vi "I2C Write Reg Block.vi"(8 "error in (no error)":errorcluster, 9 "Values":u8[](array[numeric]), 10 "Register":i32, 11 "I2C Device":T1) -> (0 "error out":errorcluster, 3 "I2C Device out":T1)   [LabVIEW 2020, in "wiringPi.lvlib"]
doc: "<b>_______________________________________________________________</b>\n** Author: Juan José Villacorta\n** LabVIEW wrapper for C library <b> wiringPi </b>,\n** https://github.com/WiringPi/WiringPi\n<b>_______________________________________________________________</b>\n/*\n * Write a block of data to a register on the device\n**********************************************************************************\n*/"
uses:
  wiringPi.lvlib
  Type Defs/I2C Device.ctl
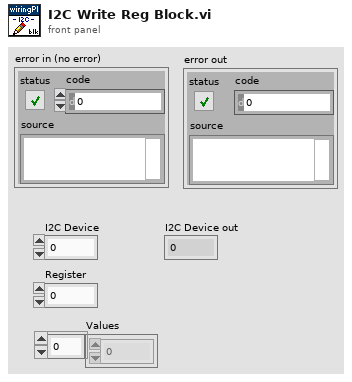
[diagram p1: front panel]
types:
  T1 = typedef "wiringPi.lvlib/I2C Device.ctl" = i32
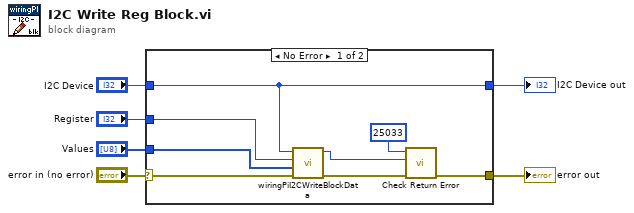
[diagram p0: block diagram]
diagram:
  n1 = case shown="No Error" "error in (no error)" {
    selector: "error in (no error)" -> [w13 w16]
    tunnel: [w14 w16] -> w5
    tunnel: "I2C Device" -> [w11 w15]
    tunnel: [w11 w15] -> w4
    tunnel: "Register" -> [w8 _]
    tunnel: "Values" -> [w7 _]
    frame No Error {
      n2 = call "wiringPiI2CWriteBlockData.vi"("error in (no error)"=w13, "values"=w7, "reg"=w8, "devID"=w11) -> ("error out"=w12:errorcluster, "return"=w10:i32)  [unwired: 6 in]
      n3 = call "Check Return Error.vi"("error in (no error)"=w12, "Return code"=w10, "Error number"=25033) -> ("error out"=w14:errorcluster)  [unwired: 8 in]
    }
    frame Error {
    }
  }
  "error out" <- w5
  "I2C Device out" <- w4
